vi "Lookup Bool.vi"(8 "error in":errorcluster, 10 "name":string, 11 "bool values":cluster{"name":string, "on":bool}[](array[cluster])) -> (0 "error out":errorcluster, 2 "found":bool, 3 "on":bool)   [LabVIEW 2026]
doc: "Finds the first boolean IO value with the given name. Linear search, exact match, case-sensitive. Outputs the value and whether it was found."
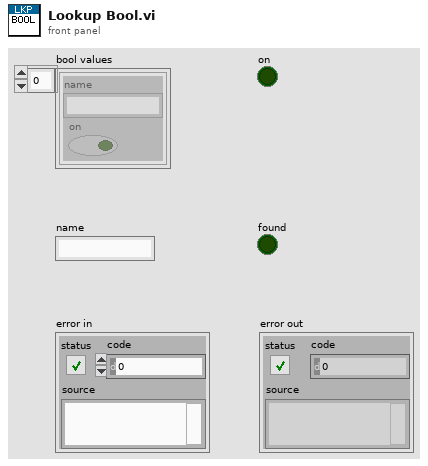
[diagram p1: front panel]
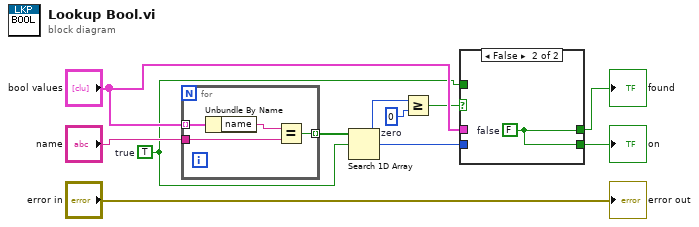
[diagram p0: block diagram]
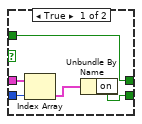
[diagram p2: hidden frame]
diagram:
  w8 = 0  # zero
  w5 = TRUE  # true
  n1 = for {
    tunnel: "bool values" -> [w14] mode=indexing
    tunnel: "name" -> [w12]
    tunnel: [w11] -> w9 mode=indexing
    n2 = Unbundle By Name(w14) -> ("name"=w13:string)
    n3 = Equal?(x=w13, y=w12) -> (x = y?=w11:bool)
  }
  n4 = Search 1D Array(1D array=w9, element=w5) -> (index of element=w7:i32)  [unwired: 1 in]
  n5 = Greater Or Equal?(x=w7, y=w8) -> (x >= y?=w4:bool)
  n6 = case shown="False" w4 {
    tunnel: w7 -> [w19 _]
    tunnel: "bool values" -> [w18 _]
    tunnel: [w16 w20] -> w3
    tunnel: [w15 w20] -> w2
    tunnel: w5 -> [w15 _]
    frame True {
      n7 = Index Array(array=w18, index=w19) -> (element=w17:cluster{"name":string, "on":bool})
      n8 = Unbundle By Name(w17) -> ("on"=w16:bool)
    }
    frame False {
      w20 = FALSE  # false
    }
  }
  "on" <- w3
  "found" <- w2
  "error out" <- "error in"
